vi "MOKO_Plugin_First.vi"() -> ()   [LabVIEW 2018]
uses:
  Lib/STM/ExPlugin/MOKO_ExPlugin_ExPlugin_STM.ctl
  Lib/STM/ExPlugin/MOKO_ExPlugin_ExPlugin_ITEM.ctl
  Lib/STM/Loop/MOKO_ExPlugin_Loop_STM.ctl
  Lib/STM/Loop/MOKO_ExPlugin_Loop_ITEM.ctl
  Lib/STM/Grafic/MOKO_ExPlugin_Grafic_STM.ctl
  Lib/STM/Grafic/MOKO_ExPlugin_Grafic_ITEM.ctl
panel:
  in  "Base64 String":string
  out "Screenshot indicator":bool
  in  "Screenshot":bool
  out "ExPluginStatus":bool
  out "MOKO_ExPlugin":refnum<queue>
  in  "Tab Control":enum32{"Main", "Graph", "Info"}(tab)
  in  "String":string
  in  "calculate":bool
  out "Led event":bool
  out "Led loop":bool
  in  "Change Led loop":bool
  in  "Open SubVi":bool
  in  "Number1":dbl caption="Число 1"
  in  "Number2":dbl caption="Число 2"
  out "Sum":dbl caption="Сумма"
  in  "Stop Graph":bool
  in  "Start grafic":bool caption="Start"
  in  "Reset":bool
  out "Waveform Graph":dbl[](graph)
  # "Led indicators"
  # "Summ"
  # "+"
  # "="
  # "Данный плагин предназначен для демонстрации возможностей программы \nMOKO SE, а также является шаблоном для разработки собственных плагинов.\n\nExPlugin делится на 3 части: *Main*, *Graph*, *Info*, каждая из которых имеет \nсвою функциональность."
  # "Main"
  # "В окне *Main* реализовапны функции *ChangeLedLoop*, *String*, *Number1*,\n*Number2* и *Sum*. Каждая функция, кроме *Sum*, работает в режиме *set*. \nФункция *Sum* работает в режиме *Get*  и возвращает значение типа string. \nФункция *String* работает в режимах *get* и *set*."
  # "Graph"
  # "В окне *Graph* реализован график и функции управления им. Все функции \nработают в режиме *set*."
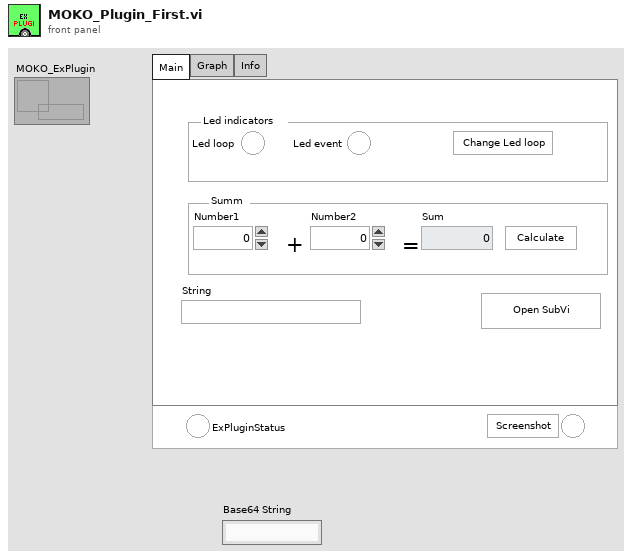
[diagram p1: front panel]
types:
  T1 = typedef "MOKO_ExPlugin_Loop_STM.ctl" = cluster{"main stm":T2, "data":string}
  T2 = typedef "MOKO_ExPlugin_Loop_ITEM.ctl" = enum16{"idle", "_____ main_____ ", "Stop", "OpenSubVi", "ScreenShot", "_____SUM _____", "Sum", "_____Settings_____", "Led"}
  T3 = typedef "MOKO_ExPlugin_Grafic_STM.ctl" = cluster{"main stm":T4, "data":string}
  T4 = typedef "MOKO_ExPlugin_Grafic_ITEM.ctl" = enum16{"idle", "Write Graph", "Reset", "Start", "Stop", "Stop Graph", "Screenshot"}
  T5 = typedef "MOKO_ExPlugin_ExPlugin_STM.ctl" = cluster{"main stm":T6, "data":string}
  T6 = typedef "MOKO_ExPlugin_ExPlugin_ITEM.ctl" = enum16{"idle", "ExPlugin read", "ExPlugin write"}
  T7 = typedef "imagedata.ctl" = cluster{"image type":i32, "image depth":i32, "image":u8[], "mask":u8[], "colors":u32[], "Rectangle":cluster{"left":i16, "top":i16, "right":i16, "bottom":i16}}
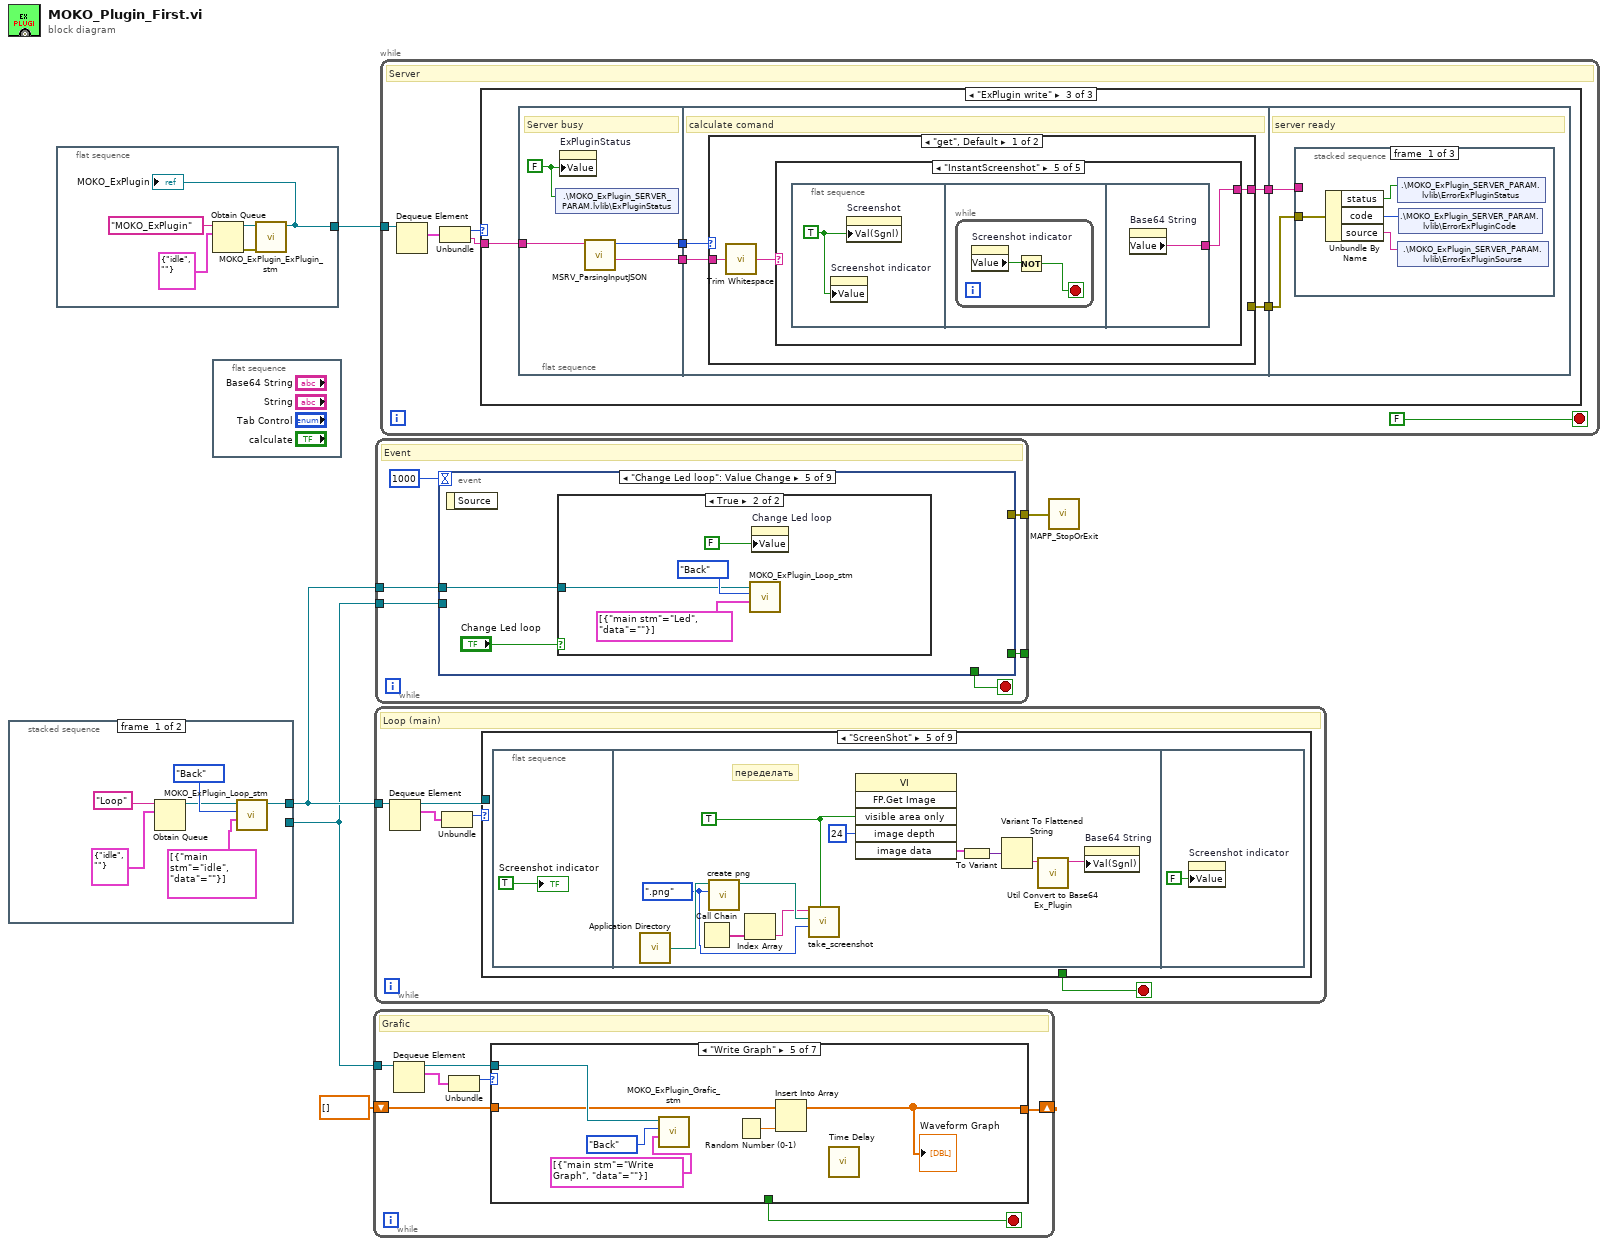
[diagram p0: block diagram]
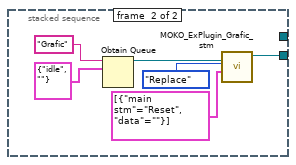
[diagram p2: hidden frame]
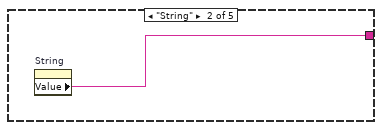
[diagram p6: hidden frame]
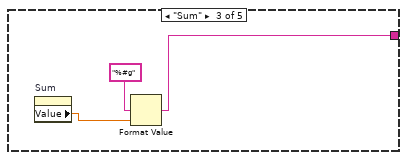
[diagram p7: hidden frame]
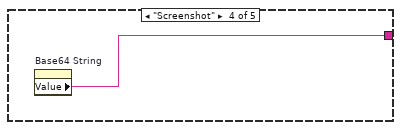
[diagram p8: hidden frame]
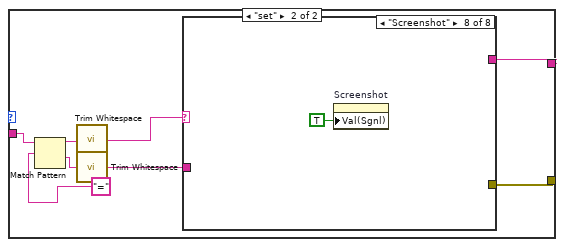
[diagram p9: hidden frame]
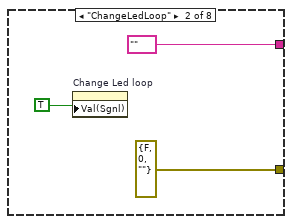
[diagram p11: hidden frame]
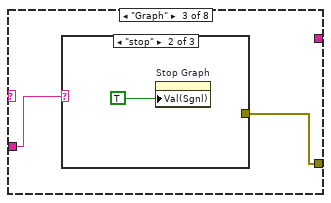
[diagram p12: hidden frame]
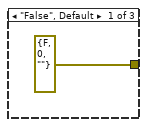
[diagram p13: hidden frame]
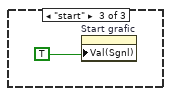
[diagram p14: hidden frame]
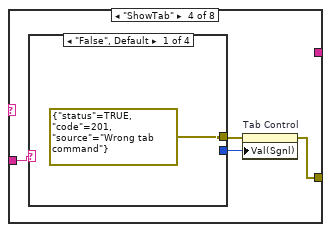
[diagram p15: hidden frame]
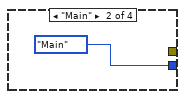
[diagram p16: hidden frame]
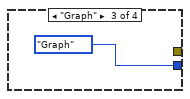
[diagram p17: hidden frame]
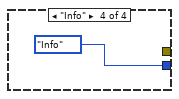
[diagram p18: hidden frame]
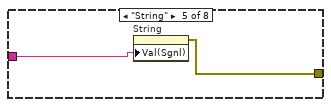
[diagram p19: hidden frame]
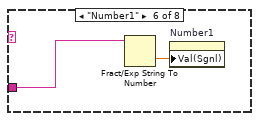
[diagram p20: hidden frame]
diagram:
  n1 = stacked-sequence {
    tunnel: [w6 _] -> w3
    tunnel: [_ w12] -> w1
    frame #0 {
      n2 = Obtain Queue(name (unnamed)="Loop", element data type=T1 {"main stm"=enum."idle", "data"=""} ("MOKO_SE_STM")) -> (queue out=w8:refnum<queue>)  [unwired: 3 in, 2 out]
      n3 = call "MOKO_ExPlugin_Loop_stm.vi"("StateMachineSteps"=T1[] [{"main stm"=enum."idle", "data"=""}], "FNs"=enum16{"Back", "Front", "Replace"}."Back", "queue in"=w8) -> ("queue out"=w6:refnum<queue>)  [unwired: 7 in, 1 out]
    }
    frame #1 {
      n4 = Obtain Queue(name (unnamed)="Grafic", element data type=T3 {"main stm"=enum."idle", "data"=""} ("MOKO_NMEA")) -> (queue out=w17:refnum<queue>)  [unwired: 3 in, 2 out]
      n5 = call "MOKO_ExPlugin_Grafic_stm.vi"("StateMachineSteps"=T3[] [{"main stm"=enum."Reset", "data"=""}], "FNs"=enum16{"Back", "Front", "Replace"}."Replace", "queue in"=w17) -> ("queue out"=w12:refnum<queue>)  [unwired: 7 in, 1 out]
    }
  }
  n6 = flat-sequence {
    tunnel: [w18] -> w4
    frame #0 {
      n7 = Obtain Queue(name (unnamed)="MOKO_ExPlugin", element data type=T5 {"main stm"=enum."idle", "data"=""} ("MOKO_SE_STM")) -> (queue out=w20:refnum<queue>, error out=w19:errorcluster)  [unwired: 3 in, 1 out]
      n8 = call "MOKO_ExPlugin_ExPlugin_stm.vi"("error in"=w19, "queue in"=w20) -> ("queue out"=w18:refnum<queue>)  [unwired: 8 in, 1 out]
      "MOKO_ExPlugin" <- w18
    }
  }
  n9 = flat-sequence {
    frame #0 {
    }
  }
  n10 = while {
    tunnel: w1 -> [w28]
    shift-right: [w26] -> _
    shift-left: dbl[] [] ("Waveform Graph") -> [w27]
    stop <- w25 stop-if-true
    # "Grafic"
    n11 = Dequeue Element(queue=w28) -> (queue out=w29:refnum<queue>, element=w24:T3)  [unwired: 2 in, 2 out]
    n12 = Unbundle(w24) -> ("main stm"=w23:T4)  [unwired: 1 out]
    n13 = case shown="\"Write Graph\"" w23 {
      tunnel: w29 -> [_ w34 w35 _ w45 _ _]
      tunnel: w27 -> [w30 w31 w38 w40 w43 _ w48]
      tunnel: [w30 w31 w38 w40 w41 w47 w48] -> w26
      tunnel: [_ _ _ TRUE _ _ _] -> w25
      frame "idle", Default {
      }
      frame "Start" {
        n14 = call "MOKO_ExPlugin_Grafic_stm.vi"("StateMachineSteps"=T3[] [{"main stm"=enum."Write Graph", "data"=""}], "FNs"=enum16{"Back", "Front", "Replace"}."Front", "queue in"=w34) -> ()  [unwired: 7 in, 2 out]
      }
      frame "Stop Graph" {
        n15 = call "MOKO_ExPlugin_Grafic_stm.vi"("StateMachineSteps"=T3[] [{"main stm"=enum."idle", "data"=""}], "FNs"=enum16{"Back", "Front", "Replace"}."Replace", "queue in"=w35) -> ()  [unwired: 7 in, 2 out]
      }
      frame "Stop" {
      }
      frame "Write Graph" {
        n16 = call "MOKO_ExPlugin_Grafic_stm.vi"("StateMachineSteps"=T3[] [{"main stm"=enum."Write Graph", "data"=""}], "FNs"=enum16{"Back", "Front", "Replace"}."Back", "queue in"=w45) -> ()  [unwired: 7 in, 2 out]
        n17 = Random Number (0-1)() -> (number: 0 to 1=w42:dbl)
        n18 = Insert Into Array(array=w43, new element=w42) -> (w41:dbl[])  [unwired: 1 in]
        "Waveform Graph" <- w41
        n19 = call "Time Delay"() -> ()  [unwired: 11 in, 1 out]
      }
      frame "Reset" {
        w47 = dbl[] [] ("Waveform Graph")
        n20 = property on="Waveform Graph" class="WFGraph (strict)"("Value"=w47) -> ()  [unwired: 2 in, 2 out]
      }
      frame "Screenshot" {
      }
    }
  }
  n21 = while {
    tunnel: w3 -> [w53]
    stop <- w51 stop-if-true
    # "Loop (main)"
    n22 = Dequeue Element(queue=w53) -> (queue out=w52:refnum<queue>, element=w50:T1)  [unwired: 2 in, 2 out]
    n23 = Unbundle(w50) -> ("main stm"=w49:T2)  [unwired: 1 out]
    n24 = case shown="\"ScreenShot\"" w49 {
      selector: w49 -> [_ _ _ w55 _ _ _ _ _]
      tunnel: w52 -> [_ _ _ _ _ _ _ _ _]
      tunnel: [_ _ TRUE _ _ _ _ _ _] -> w51
      frame "idle", Default {
      }
      frame "_____ main_____ " {
      }
      frame "Stop" {
      }
      frame "OpenSubVi" {
        n25 = flat-sequence {
          tunnel: w55 -> [_]
          frame #0 {
            n26 = call "ExSubVi.vi"() -> ()  [unwired: 12 in]
          }
        }
      }
      frame "ScreenShot" {
        n27 = flat-sequence {
          frame #0 {
            "Screenshot indicator" <- TRUE
          }
          frame #1 {
            w61 = TRUE ("Visible Area Only")
            w65 = enum32{".png", ".jpg", ".bmp"}.".png" ("IMG_FORMAT")
            # "переделать"
            n28 = call <vilib>:"Application Directory.vi"() -> ("Application Directory"=w67:path)
            n29 = Call Chain() -> (call chain=w64:string[])
            n30 = call "create png.vi"("IMG_FORMAT"=w65, "base path"=w67) -> ("path"=w66:path)  [unwired: 8 in, 1 out]
            n31 = Index Array(array=w64) -> (element=w63:string)  [unwired: 1 in]
            n32 = call "take_screenshot.vi"("Visible area only? (f)"=w61, "IMG_FORMAT"=w65, "Image path"=w66, "vi path"=w63) -> ()  [unwired: 3 in, 2 out]
            n33 = invoke class="VI" method="FP.Get Image"("visible area only"=w61, "image depth"=24 ("Image Depth")) -> ("image data"=w59:T7)  [unwired: 4 in, 5 out]
            n34 = To Variant(anything=w59) -> (Variant=w60:variant)
            n35 = Variant To Flattened String(Variant=w60) -> (data string=w58:string)  [unwired: 1 out]
            n36 = call "Util Convert to Base64 Ex_Plugin.vi"("String"=w58) -> ("Base64 String"=w57:string)  [unwired: 10 in]
            n37 = property on="Base64 String" class="Str"("Val(Sgnl)"=w57) -> ()  [unwired: 2 in, 2 out]
          }
          frame #2 {
            n38 = property on="Screenshot indicator" class="Bool (strict)"("Value"=FALSE) -> ()  [unwired: 2 in, 2 out]
          }
        }
      }
      frame "_____SUM _____" {
      }
      frame "Sum" {
        n39 = property on="Number2" class="DigNum (strict)"() -> ("Value"=w71:dbl)  [unwired: 2 in, 2 out]
        n40 = property on="Number1" class="DigNum (strict)"() -> ("Value"=w70:dbl)  [unwired: 2 in, 2 out]
        n41 = Add(x=w70, y=w71) -> (x+y=→"Sum":dbl)
      }
      frame "_____Settings_____" {
      }
      frame "Led" {
        n42 = property on="Led loop" class="Bool (strict)"() -> ("Value"=w73:bool)  [unwired: 2 in, 2 out]
        n43 = Not(x=w73) -> (.not. x?=→"Led loop":bool)
      }
    }
  }
  n44 = while {
    tunnel: w3 -> [w78]
    tunnel: w1 -> [w77]
    tunnel: [w75] -> _
    tunnel: [w74] -> w2
    stop <- w76 stop-if-true
    # "Event"
    n45 = event shown="[4] \"Change Led loop\": Value Change" {
      selector: _ -> [_ _ _ _ _ _ _ _ _]
      dyn-events: _ -> [_ _ _ _ _ _ _ _ _]
      timeout: 1000 -> [_ _ _ _ _ _ _ _ _]
      tunnel: w78 -> [w80 _ w92 w96 w100 w107 _ _ w114]
      tunnel: w77 -> [_ w87 w95 _ _ _ w110 w113 _]
      tunnel: [_ _ w89 _ _ _ _ _ _] -> w76
      tunnel: [_ _ w89 _ _ _ _ _ _] -> w75
      tunnel: [_ _ errorcluster {"status"=FALSE, "code"=0, "source"=""} ("Error In") _ _ _ _ _ _] -> w74
      event Timeout {
        n46 = event-data() -> ()  [unwired: 1 in, 3 out]
        n47 = property on="Led event" class="Bool (strict)"() -> ("Value"=w84:bool)  [unwired: 2 in, 2 out]
        n48 = Not(x=w84) -> (.not. x?=→"Led event":bool)
        n49 = call "MOKO_ExPlugin_Loop_stm.vi"("StateMachineSteps"=T1[] [{"main stm"=enum."Led", "data"=""}], "FNs"=enum16{"Back", "Front", "Replace"}."Back", "queue in"=w80) -> ()  [unwired: 7 in, 2 out]
      }
      event "Start grafic": Value Change {
        n50 = event-data() -> ()  [unwired: 1 in, 6 out]
        n51 = call "MOKO_ExPlugin_Grafic_stm.vi"("StateMachineSteps"=T3[] [{"main stm"=enum."Start", "data"=""}], "FNs"=enum16{"Back", "Front", "Replace"}."Front", "queue in"=w87) -> ()  [unwired: 7 in, 2 out]
      }
      event Panel Close {
        w89 = TRUE
        n52 = event-data() -> ()  [unwired: 1 in, 4 out]
        n53 = call "MOKO_ExPlugin_Loop_stm.vi"("StateMachineSteps"=T1[] [{"main stm"=enum."Stop", "data"=""}], "FNs"=enum16{"Back", "Front", "Replace"}."Replace", "queue in"=w92) -> ()  [unwired: 7 in, 2 out]
        n54 = call "MOKO_ExPlugin_Grafic_stm.vi"("StateMachineSteps"=T3[] [{"main stm"=enum."Stop", "data"=""}], "FNs"=enum16{"Back", "Front", "Replace"}."Replace", "queue in"=w95) -> ()  [unwired: 7 in, 2 out]
      }
      event "Number1", "Number2": Value Change {
        n55 = event-data() -> ()  [unwired: 1 in, 6 out]
        n56 = call "MOKO_ExPlugin_Loop_stm.vi"("StateMachineSteps"=T1[] [{"main stm"=enum."Sum", "data"=""}], "FNs"=enum16{"Back", "Front", "Replace"}."Back", "queue in"=w96) -> ()  [unwired: 7 in, 2 out]
      }
      event "Change Led loop": Value Change {
        n57 = event-data() -> ()  [unwired: 1 in, 1 out]
        n58 = case shown="True" "Change Led loop" {
          tunnel: w100 -> [_ w102]
          frame False {
          }
          frame True {
            n59 = call "MOKO_ExPlugin_Loop_stm.vi"("StateMachineSteps"=T1[] [{"main stm"=enum."Led", "data"=""}], "FNs"=enum16{"Back", "Front", "Replace"}."Back", "queue in"=w102) -> ()  [unwired: 7 in, 2 out]
            n60 = property on="Change Led loop" class="Bool (strict)"("Value"=FALSE ("Change Led loop")) -> ()  [unwired: 2 in, 2 out]
          }
        }
      }
      event "Open SubVi": Value Change {
        n61 = event-data() -> ()  [unwired: 1 in, 6 out]
        n62 = call "MOKO_ExPlugin_Loop_stm.vi"("StateMachineSteps"=T1[] [{"main stm"=enum."OpenSubVi", "data"=""}], "FNs"=enum16{"Back", "Front", "Replace"}."Back", "queue in"=w107) -> ()  [unwired: 7 in, 2 out]
      }
      event "Stop Graph": Value Change {
        n63 = event-data() -> ()  [unwired: 1 in, 6 out]
        n64 = call "MOKO_ExPlugin_Grafic_stm.vi"("StateMachineSteps"=T3[] [{"main stm"=enum."Stop Graph", "data"=""}], "FNs"=enum16{"Back", "Front", "Replace"}."Replace", "queue in"=w110) -> ()  [unwired: 7 in, 2 out]
      }
      event "Reset": Value Change {
        n65 = event-data() -> ()  [unwired: 1 in, 6 out]
        n66 = call "MOKO_ExPlugin_Grafic_stm.vi"("StateMachineSteps"=T3[] [{"main stm"=enum."Reset", "data"=""}], "FNs"=enum16{"Back", "Front", "Replace"}."Front", "queue in"=w113) -> ()  [unwired: 7 in, 2 out]
      }
      event "Screenshot": Value Change {
        n67 = event-data() -> ()  [unwired: 1 in, 1 out]
        n68 = call "MOKO_ExPlugin_Loop_stm.vi"("StateMachineSteps"=T1[] [{"main stm"=enum."ScreenShot", "data"=""}], "FNs"=enum16{"Back", "Front", "Replace"}."Back", "queue in"=w114) -> ()  [unwired: 7 in, 2 out]
      }
    }
  }
  n69 = while {
    tunnel: w4 -> [w120]
    stop <- FALSE stop-if-true
    # "Server"
    n70 = Dequeue Element(queue=w120) -> (element=w119:T5)  [unwired: 2 in, 3 out]
    n71 = Unbundle(w119) -> ("main stm"=w118:T6, "data"=w117:string)
    n72 = case shown="\"ExPlugin write\"" w118 {
      tunnel: w117 -> [_ _ w124]
      frame "idle", Default {
      }
      frame "ExPlugin read" {
      }
      frame "ExPlugin write" {
        n73 = flat-sequence {
          tunnel: w124 -> [w129]
          tunnel: [w128] -> w123
          tunnel: [w127] -> w122
          tunnel: [w131] -> w126
          tunnel: [w134] -> w125
          tunnel: w123 -> [w133]
          tunnel: w122 -> [w132]
          tunnel: w126 -> [w180]
          tunnel: w125 -> [w179]
          frame #0 {
            w130 = FALSE
            # "Server busy"
            n74 = shared-variable ".\\MOKO_ExPlugin_SERVER_PARAM.lvlib\\ExPluginStatus"(w130) -> ()  [unwired: 1 in, 1 out]
            n75 = property on="ExPluginStatus" class="Bool (strict)"("Value"=w130) -> ()  [unwired: 2 in, 2 out]
            n76 = call "MSRV_ParsingInputJSON.vi"("data"=w129) -> ("command"=w127:string, "Mode out"=w128:enum16{"get", "set", "close", "Init", "Check"})  [unwired: 7 in, 2 out]
          }
          frame #1 {
            # "calculate comand"
            n77 = case shown="\"get\", Default" w133 {
              tunnel: [_ w155] -> w134
              tunnel: w132 -> [w137 w153]
              tunnel: [w135 w148] -> w131
              frame "get", Default {
                n78 = call <vilib>:"Trim Whitespace.vi"("string"=w137) -> ("trimmed string"=w136:string)  [unwired: 1 in]
                n79 = case shown="\"InstantScreenshot\"" w136 {
                  tunnel: [_ w138 w140 w142 w143] -> w135
                  frame "False", Default {
                  }
                  frame "String" {
                    n80 = property on="String" class="Str"() -> ("Value"=w138:string)  [unwired: 2 in, 2 out]
                  }
                  frame "Sum" {
                    n81 = property on="Sum" class="DigNum (strict)"() -> ("Value"=w139:dbl)  [unwired: 2 in, 2 out]
                    n82 = Format Value(format string="%#g", value (0)=w139) -> (output string=w140:string)  [unwired: 1 in]
                  }
                  frame "Screenshot" {
                    n83 = property on="Base64 String" class="Str"() -> ("Value"=w142:string)  [unwired: 2 in, 2 out]
                  }
                  frame "InstantScreenshot" {
                    n84 = flat-sequence {
                      tunnel: [w147] -> w143
                      frame #0 {
                        w144 = TRUE ("Value (Signaling)")
                        n85 = property on="Screenshot indicator" class="Bool (strict)"("Value"=w144) -> ()  [unwired: 2 in, 2 out]
                        n86 = property on="Screenshot" class="Bool (strict)"("Val(Sgnl)"=w144) -> ()  [unwired: 2 in, 2 out]
                      }
                      frame #1 {
                        n87 = while {
                          stop <- w145 stop-if-true
                          n88 = property on="Screenshot indicator" class="Bool (strict)"() -> ("Value"=w146:bool)  [unwired: 2 in, 2 out]
                          n89 = Not(x=w146) -> (.not. x?=w145:bool)
                        }
                      }
                      frame #2 {
                        n90 = property on="Base64 String" class="Str"() -> ("Value"=w147:string)  [unwired: 2 in, 2 out]
                      }
                    }
                  }
                }
              }
              frame "set" {
                n91 = Match Pattern(string=w153, regular expression="=") -> (before substring=w151:string, after substring=w154:string)  [unwired: 1 in, 2 out]
                n92 = call <vilib>:"Trim Whitespace.vi"("string"=w151) -> ("trimmed string"=w150:string)  [unwired: 1 in]
                n93 = call <vilib>:"Trim Whitespace.vi"("string"=w154) -> ("trimmed string"=w149:string)  [unwired: 1 in]
                n94 = case shown="\"Screenshot\"" w150 {
                  tunnel: [_ errorcluster {"status"=FALSE, "code"=0, "source"=""} ("error out") w159 w166 w172 _ _ _] -> w155
                  tunnel: w149 -> [_ _ w160 w167 w173 w174 w176 _]
                  tunnel: [_ "" _ _ _ _ _ _] -> w148
                  frame "False", Default {
                  }
                  frame "ChangeLedLoop" {
                    n95 = property on="Change Led loop" class="Bool (strict)"("Val(Sgnl)"=TRUE) -> ()  [unwired: 2 in, 2 out]
                  }
                  frame "Graph" {
                    n96 = case shown="\"stop\"" w160 {
                      tunnel: [errorcluster {"status"=FALSE, "code"=0, "source"=""} ("error constant") _ _] -> w159
                      frame "False", Default {
                      }
                      frame "stop" {
                        n97 = property on="Stop Graph" class="Bool (strict)"("Val(Sgnl)"=TRUE) -> ()  [unwired: 2 in, 2 out]
                      }
                      frame "start" {
                        n98 = property on="Start grafic" class="Bool (strict)"("Val(Sgnl)"=TRUE) -> ()  [unwired: 2 in, 2 out]
                      }
                    }
                  }
                  frame "ShowTab" {
                    n99 = case shown="\"False\", Default" w167 {
                      tunnel: [errorcluster {"status"=TRUE, "code"=201, "source"="Wrong tab command"} ("error in (no error)") _ _ _] -> w165
                      tunnel: [_ enum32{"Main", "Graph", "Info"}."Main" ("Value (Signaling)") enum32{"Main", "Graph", "Info"}."Graph" ("Value (Signaling)") enum32{"Main", "Graph", "Info"}."Info" ("Value (Signaling)")] -> w164
                      frame "False", Default {
                      }
                      frame "Main" {
                      }
                      frame "Graph" {
                      }
                      frame "Info" {
                      }
                    }
                    n100 = property on="Tab Control" class="TabCtl (strict)"(error in=w165, "Val(Sgnl)"=w164) -> (error out=w166:errorcluster)  [unwired: 1 in, 1 out]
                  }
                  frame "String" {
                    n101 = property on="String" class="Str"("Val(Sgnl)"=w173) -> (error out=w172:errorcluster)  [unwired: 2 in, 1 out]
                  }
                  frame "Number1" {
                    n102 = Fract/Exp String To Number(string=w174) -> (number=w175:dbl)  [unwired: 3 in, 1 out]
                    n103 = property on="Number1" class="DigNum (strict)"("Val(Sgnl)"=w175) -> ()  [unwired: 2 in, 2 out]
                  }
                  frame "Number2" {
                    n104 = Fract/Exp String To Number(string=w176) -> (number=w177:dbl)  [unwired: 3 in, 1 out]
                    n105 = property on="Number2" class="DigNum (strict)"("Val(Sgnl)"=w177) -> ()  [unwired: 2 in, 2 out]
                  }
                  frame "Screenshot" {
                    n106 = property on="Screenshot" class="Bool (strict)"("Val(Sgnl)"=TRUE ("Value (Signaling)")) -> ()  [unwired: 2 in, 2 out]
                  }
                }
              }
            }
          }
          frame #2 {
            # "server ready"
            n107 = stacked-sequence {
              tunnel: w180 -> [_ w185 _]
              tunnel: w179 -> [w181 _ _]
              frame #0 {
                n108 = Unbundle By Name(w181) -> ("status"=w182:bool, "code"=w183:i32, "source"=w184:string)
                n109 = shared-variable ".\\MOKO_ExPlugin_SERVER_PARAM.lvlib\\ErrorExPluginStatus"(w182) -> ()  [unwired: 1 in, 1 out]
                n110 = shared-variable ".\\MOKO_ExPlugin_SERVER_PARAM.lvlib\\ErrorExPluginSourse"(w184) -> ()  [unwired: 1 in, 1 out]
                n111 = shared-variable ".\\MOKO_ExPlugin_SERVER_PARAM.lvlib\\ErrorExPluginCode"(w183) -> ()  [unwired: 1 in, 1 out]
              }
              frame #1 {
                n112 = shared-variable ".\\MOKO_ExPlugin_SERVER_PARAM.lvlib\\ExPluginData"(w185) -> ()  [unwired: 1 in, 1 out]
              }
              frame #2 {
                w186 = TRUE
                n113 = shared-variable ".\\MOKO_ExPlugin_SERVER_PARAM.lvlib\\ExPluginStatus"(w186) -> ()  [unwired: 1 in, 1 out]
                "ExPluginStatus" <- w186
              }
            }
          }
        }
      }
    }
  }
  n114 = call "MAPP_StopOrExit.vi"("Error In"=w2) -> ()
